vi "AIT 664 - Conditionally Serialize.vi"(8 "error in (no error)":errorcluster, 11 "Device Item Ref in":T1 format="%.0x") -> (0 "error out":errorcluster)   [LabVIEW 2015, in "AIT 664 Custom Device.lvlib"]
uses:
  AIT 664 Custom Device.lvlib
  <vilib>/NI Veristand/Custom Device API/Custom Device Item Ref.ctl
  <vilib>/NI Veristand/Custom Device API/NI VeriStand - Add Custom Device Dependencies.vi
  <vilib>/NI Veristand/Custom Device API/NI VeriStand - Reset Custom Device Dependencies.vi
  <vilib>/NI Veristand/Custom Device API/Get Item Property (Boolean).vi
  <vilib>/NI Veristand/Custom Device API/Get Item Property (Path).vi
  Controls and Global/Global.vi
  <vilib>/NI Veristand/Custom Device API/Custom Device API.lvlib
panel:
  out "Destination File":path
  out "Converted File":path
  out "Value":path
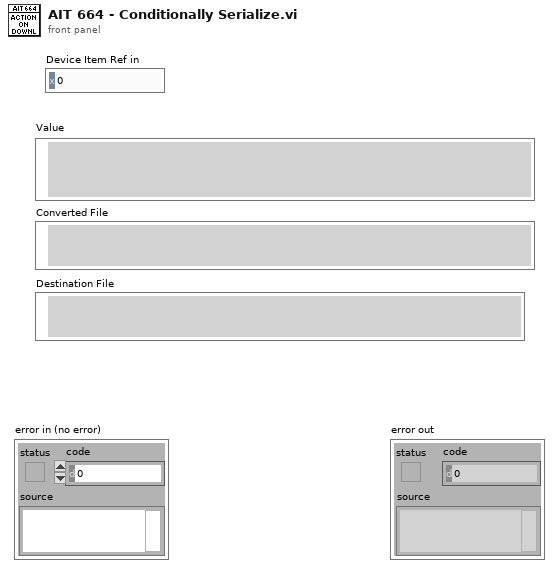
[diagram p1: front panel]
types:
  T1 = typedef "Custom Device API.lvlib/Custom Device Item Ref.ctl" = u64
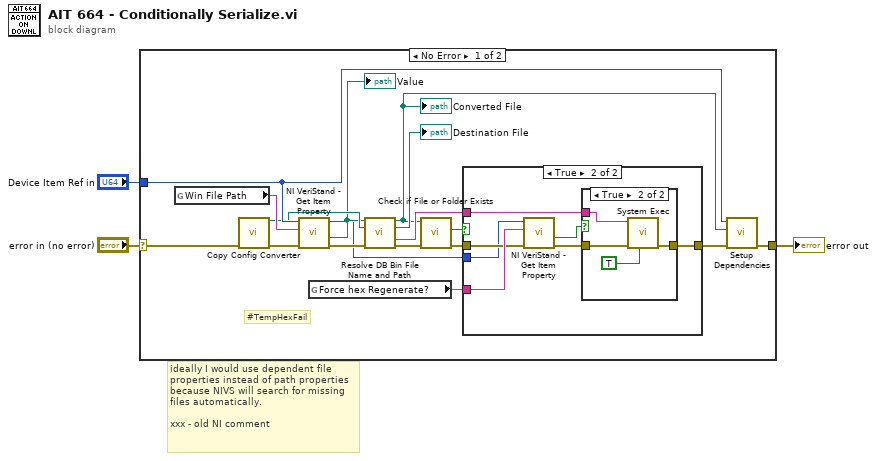
[diagram p0: block diagram]
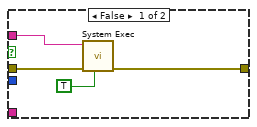
[diagram p2: hidden frame]
diagram:
  # "ideally I would use dependent file properties instead of path properties because NIVS will search for missing files automatically.\n\nxxx - old NI comment"
  n1 = case shown="No Error" "error in (no error)" {
    selector: "error in (no error)" -> [w14 w37]
    tunnel: [w11 w37] -> w2
    tunnel: "Device Item Ref in" -> [w15 _]
    frame No Error {
      # "#TempHexFail"
      n2 = global read "Global.vi" "Win File Path"() -> (w20:string)
      n3 = call "Copy Config Converter.vi"("error in (no error)"=w14) -> ("path"=w13:path, "error out"=w16:errorcluster)  [unwired: 13 in]
      n4 = call-poly <vilib>:"NI VeriStand - Get Item Property.vi"("error in (no error)"=w16, "Property Name"=w20, "Item Ref in"=w15) -> ("error out"=w19:errorcluster, "Value"=w12:path, "Item Ref out"=w8:T1)  [unwired: 5 in, 1 out]
      "Value" <- w12
      n5 = global read "Global.vi" "Force hex Regenerate?"() -> (w9:string)
      n6 = call "Resolve DB Bin File Name and Path.vi"("DB XML File"=w12, "Path to Tools"=w13, "error in"=w19) -> ("Converted File"=w7:path, "Destination File"=→"Destination File":path, "SysExec"=w10:string, "error out"=w5:errorcluster)  [unwired: 9 in]
      "Converted File" <- w7
      n7 = call <vilib>:"Check if File or Folder Exists.vi"("error in (no error)"=w5, "path"=w7) -> ("error out"=w4:errorcluster, "file or folder exists?"=w6:bool)  [unwired: 7 in, 1 out]
      n8 = case shown="True" w6 {
        tunnel: [w22 w31] -> w18
        tunnel: w10 -> [w21 w30]
        tunnel: w9 -> [_ w29]
        tunnel: w4 -> [w23 w28]
        tunnel: w8 -> [_ w26]
        frame False {
          n9 = call <vilib>:"System Exec.vi"("run minimized? (F)"=TRUE, "error in (no error)"=w23, "command line"=w21) -> ("error out"=w22:errorcluster)  [unwired: 5 in, 3 out]
        }
        frame True {
          n10 = call-poly <vilib>:"NI VeriStand - Get Item Property.vi"("error in (no error)"=w28, "Property Name"=w29, "Item Ref in"=w26) -> ("error out"=w27:errorcluster, "Value"=w25:bool)  [unwired: 5 in, 2 out]
          n11 = case shown="True" w25 {
            tunnel: w27 -> [w32 w35]
            tunnel: [w32 w34] -> w31
            tunnel: w30 -> [_ w33]
            frame False {
            }
            frame True {
              n12 = call <vilib>:"System Exec.vi"("run minimized? (F)"=TRUE, "error in (no error)"=w35, "command line"=w33) -> ("error out"=w34:errorcluster)  [unwired: 5 in, 3 out]
            }
          }
        }
      }
      n13 = call "Setup Dependencies.vi"("error in (no error)"=w18, "Windows Bin File"=w7, "Item Ref in"=w15) -> ("error out"=w11:errorcluster)  [unwired: 8 in]
    }
    frame Error {
    }
  }
  "error out" <- w2
